vi "Serial Port Read Simulator.vi"(2 "requested byte count":u32, 3 "port number":i32) -> (0 "error code":i32 format="%x", 1 "string read":string)   [LabVIEW 2014]
doc: "Reads the number of characters specified by <B>requested byte count</B> from the serial port indicated in <B>port number</B>."
uses:
  SimulatorGlobalOscilloscope.vi
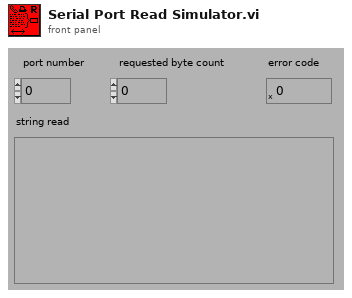
[diagram p1: front panel]
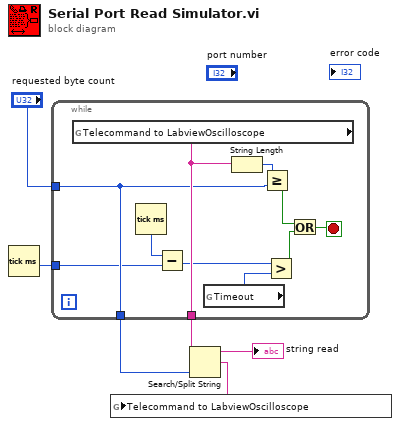
[diagram p0: block diagram]
diagram:
  n1 = Tick Count (ms)() -> (millisecond timer value=w1:u32)
  n2 = while {
    tunnel: "requested byte count" -> [w14]
    tunnel: [w15] -> w3
    tunnel: [w14] -> w2
    tunnel: w1 -> [w13]
    stop <- w11 stop-if-true
    n3 = global read "SimulatorGlobalOscilloscope.vi" "Telecommand to LabviewOscilloscope"() -> (w15:string)
    n4 = Tick Count (ms)() -> (millisecond timer value=w8:u32)
    n5 = Subtract(x=w8, y=w13) -> (x-y=w12:u32)
    n6 = global read "SimulatorGlobalOscilloscope.vi" "Timeout"() -> (w7:u16)
    n7 = String Length(string=w15) -> (length=w16:i32)
    n8 = Greater Or Equal?(x=w16, y=w14) -> (x >= y?=w10:bool)
    n9 = Greater?(x=w12, y=w7) -> (0:w9:bool)
    n10 = Or(x=w10, y=w9) -> (x .or. y?=w11:bool)
  }
  n11 = Search/Split String(string=w3, offset (0)=w2) -> (substring before match=→"string read":string, match + rest of string=w5:string)  [unwired: 1 in, 1 out]
  n12 = global write "SimulatorGlobalOscilloscope.vi" "Telecommand to LabviewOscilloscope"(w5) -> ()
